vi "Transport_Send_Command.vi"(8 "error in (no error)":errorcluster={"status"=FALSE, "code"=0, "source"="\"\""}, 10 "transport ref":string, 11 "Typed RuntimeMessage":string) -> (0 "error out":errorcluster={"status"=FALSE, "code"=0, "source"="\"\""}, 2 "status ok":bool, 3 "Send result":string)   [LabVIEW 2026]
doc: "INTENT: Send command/config/ACK requests. LOGIC: Serialize envelope with message ID/run ID and finite send deadline; record send attempts."
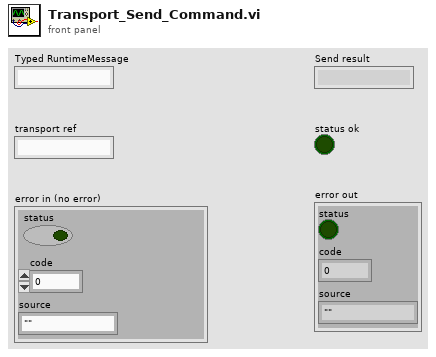
[diagram p1: front panel]
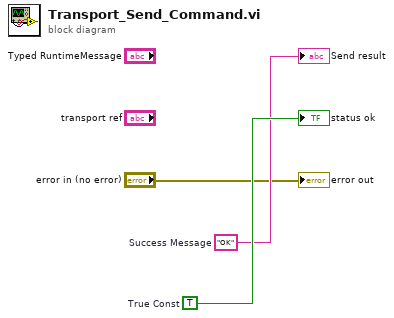
[diagram p0: block diagram]
diagram:
  w3 = TRUE  # True Const
  w2 = "OK"  # Success Message
  "Send result" <- w2
  "status ok" <- w3
  "error out" <- "error in (no error)"
